vi "script includes loader.vi"(6 "open fp?":bool=TRUE, 8 "target":i32, 9 "Plugin Search Paths":path[](array[path]), 10 "vi path (blank=new)":path, 11 "pcfg file path":path) -> (0 "error out":errorcluster)   [LabVIEW 2013]
uses:
  <vilib>/NI/Configuration Framework/class discovery singleton/class discovery singleton methods.ctl
  <vilib>/NI/Tag Bus Module Framework/root configuration/TBM configuration.lvclass
  <vilib>/NI/Configuration Framework/class discovery singleton/class discovery singleton.lvlib
  <vilib>/NI/Configuration Framework/tree serializer/NISE_CEF_TreeSerializer.lvlib
  Framework Configuration Classes/flattened data interface/PL_Serialization Interface.lvlib
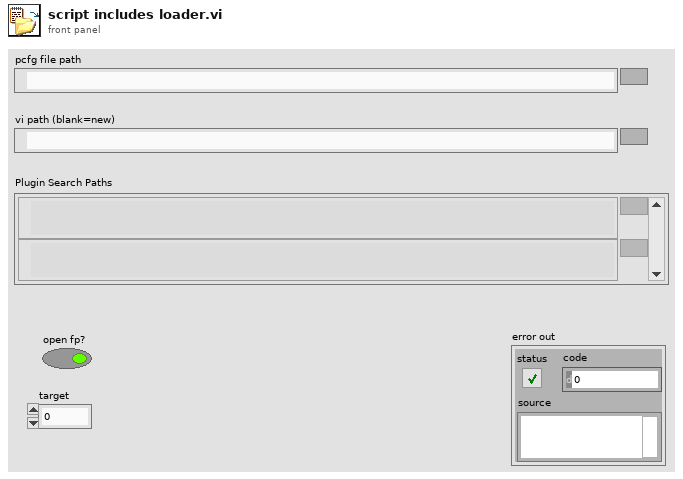
[diagram p1: front panel]
types:
  T1 = typedef "class discovery singleton.lvlib/class discovery singleton methods.ctl" = enum16{"add search paths", "load class by name", "list available classes", "get class path", "delete cache"}
  T2 = typedef "NISE_CEF_TreeSerializer.lvlib/base file format.ctl" = cluster{"version":string, "data":string}
  T3 = typedef "NISE_CEF_TreeSerializer.lvlib/flat hierarchy.ctl" = cluster{"hierarchy structure":T4, "instance data":T6[]}
  T4 = typedef "NISE_CEF_TreeSerializer.lvlib/full hierarchy.ctl" = cluster{"root":string, "hierarchy":T5[]}
  T5 = typedef "NISE_CEF_TreeSerializer.lvlib/hierarchy element.ctl" = cluster{"current node":string, "children":string[]}
  T6 = typedef "NISE_CEF_TreeSerializer.lvlib/instance data.ctl" = cluster{"ID":string, "Alias":string, "class":string, "version":string, "data":string}
  T7 = typedef "PLConfigurationSerializer.lvlib/targets cluster.ctl" = cluster{"Target Configuration":refnum<class "PL_Target Configuration.lvclass">, "engines":T8[]}
  T8 = typedef "PLConfigurationSerializer.lvlib/engines cluster.ctl" = cluster{"engine configuration":refnum<class "engine configuration.lvclass">, "modules":refnum<class "TBM module configuration.lvclass">[]}
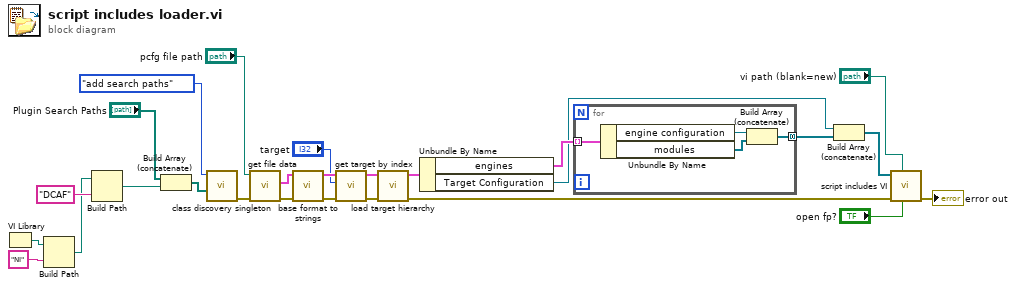
[diagram p0: block diagram]
diagram:
  n1 = VI Library() -> (path=w5:path)
  n2 = Build Path(base path=w5, name or relative path="NI") -> (appended path=w2:path)
  n3 = Build Path(base path=w2, name or relative path="DCAF") -> (appended path=w1:path)
  n4 = Build Array (concatenate)("Plugin Search Paths", w1) -> (w20:path[])
  n5 = call <vilib>:"class discovery singleton.vi"("Plugin Search Paths"=w20, "method"=class_discovery_singleton_methods."add search paths") -> ("error out"=w7:errorcluster)  [unwired: 6 in, 3 out]
  n6 = call <vilib>:"get file data.vi"("error in"=w7, "Path"="pcfg file path") -> ("error out"=w15:errorcluster, "format"=w16:T2)  [unwired: 8 in]
  n7 = call <vilib>:"base format to strings.vi"("error in"=w15, "format"=w16) -> ("error out"=w13:errorcluster, "data"=w14:T3)  [unwired: 8 in]
  n8 = call "get target by index.vi"("error in"=w13, "index"="target", "system hierarchy"=w14) -> ("error out"=w11:errorcluster, "target hierarchy"=w12:T3)  [unwired: 7 in]
  n9 = call "load target hierarchy.vi"("error in"=w11, "target hierarchy"=w12) -> ("error out"=w9:errorcluster, "targets cluster out"=w10:T7)  [unwired: 8 in]
  n10 = Unbundle By Name(w10) -> ("engines"=w25:T8[], "Target Configuration"=w23:refnum<class "PL_Target Configuration.lvclass">)
  n11 = for {
    tunnel: w25 -> [w30] mode=indexing
    tunnel: [w27] -> w24 mode=concatenating
    n12 = Unbundle By Name(w30) -> ("engine configuration"=w28:refnum<class "engine configuration.lvclass">, "modules"=w29:refnum<class "TBM module configuration.lvclass">[])
    n13 = Build Array (concatenate)(w28, w29) -> (w27:refnum<class "TBM configuration.lvclass">[])
  }
  n14 = Build Array (concatenate)(w23, w24) -> (w22:refnum<class "TBM configuration.lvclass">[])
  n15 = call "script includes VI.vi"("open fp?"="open fp?", "vi path (blank=new)"="vi path (blank=new)", "error in"=w9, "cfg objects"=w22) -> ("error out"=→"error out":errorcluster)  [unwired: 7 in]
